vi "change Queried Screenshot Data to PC File.vi"(8 "error in":errorcluster, 10 "File Path":path, 11 "VISA resource name In":refnum<visa-resource-name>) -> (0 "error out":errorcluster, 3 "VISA resource name Out":refnum<visa-resource-name>)   [LabVIEW 2023, in "Spectrum Analyzer.lvlib"]
uses:
  Spectrum Analyzer.lvlib
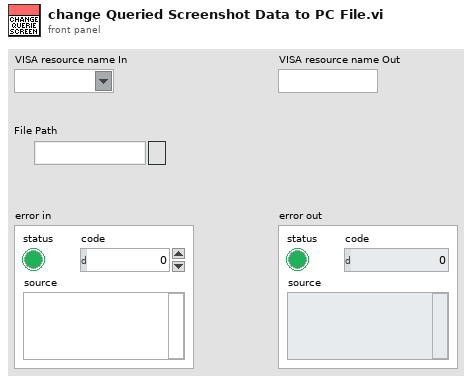
[diagram p1: front panel]
types:
  T1 = enum16{"big-endian, network order", "native, host order", "little-endian"}
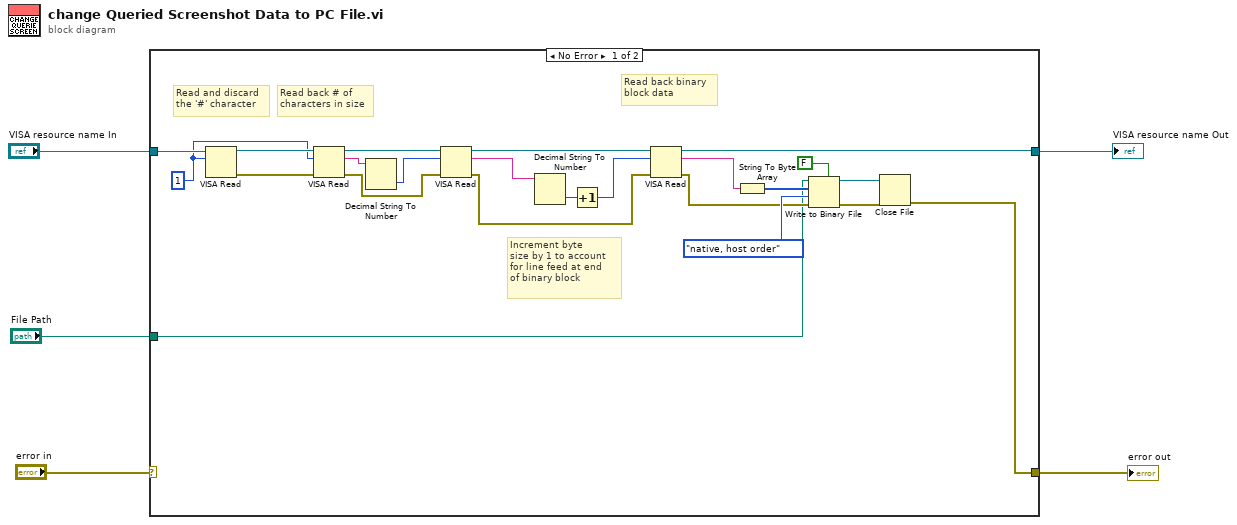
[diagram p0: block diagram]
diagram:
  n1 = case shown="No Error" "error in" {
    selector: "error in" -> [_ w30]
    tunnel: [w6 w30] -> w4
    tunnel: "VISA resource name In" -> [w11 w29]
    tunnel: [w10 w29] -> w2
    tunnel: "File Path" -> [w7 _]
    frame No Error {
      w9 = u32 1 ("byte count")
      # "Read back binary\nblock data"
      # "Increment byte\nsize by 1 to account\nfor line feed at end\nof binary block"
      # "Read back # of\ncharacters in size"
      # "Read and discard\nthe '#' character"
      n2 = VISA Read(VISA resource name=w11, byte count=w9) -> (VISA resource name out=w12:refnum<visa-resource-name>, error out=w13:errorcluster)  [unwired: 1 in, 2 out]
      n3 = VISA Read(VISA resource name=w12, byte count=w9, error in (no error)=w13) -> (VISA resource name out=w23:refnum<visa-resource-name>, read buffer=w14:string, error out=w24:errorcluster)  [unwired: 1 out]
      n4 = Decimal String To Number(string=w14) -> (number=w22:i32)  [unwired: 2 in, 1 out]
      n5 = VISA Read(VISA resource name=w23, byte count=w22, error in (no error)=w24) -> (VISA resource name out=w25:refnum<visa-resource-name>, read buffer=w26:string, error out=w28:errorcluster)  [unwired: 1 out]
      n6 = Decimal String To Number(string=w26) -> (number=w27:i32)  [unwired: 2 in, 1 out]
      n7 = Increment(x=w27) -> (x+1=w15:i32)
      n8 = VISA Read(VISA resource name=w25, byte count=w15, error in (no error)=w28) -> (VISA resource name out=w10:refnum<visa-resource-name>, read buffer=w19:string, error out=w8:errorcluster)  [unwired: 1 out]
      n9 = String To Byte Array(string=w19) -> (unsigned byte array=w20:u8[])
      n10 = Write to Binary File(file (use dialog)=w7, data=w20, error in=w8, 5:FALSE ("prepend array or string size? (T)"), 9:T1."native, host order" ("byte order (0:big-endian, network order)")) -> (refnum out=w18:refnum<file>, error out=w17:errorcluster)  [unwired: 1 in, 1 out]
      n11 = Close File(refnum=w18, error in=w17) -> (error out=w6:errorcluster)  [unwired: 1 out]
    }
    frame Error {
    }
  }
  "error out" <- w4
  "VISA resource name Out" <- w2
